vi "Set Toolbar Images.vi"(8 "error in (no error)":errorcluster, 10 "State":T3={"Buttons Displayed"=0, "Button States"=[], "Button Size"=0, "Button Style"=enum."Classic", "Active Button"=0, "Force Regen?"=FALSE, "Tip String Ref"=refnum}) -> (0 "error out":errorcluster, 2 "State Out":T3={"Buttons Displayed"=0, "Button States"=[], "Button Size"=0, "Button Style"=enum."Classic", "Active Button"=0, "Force Regen?"=FALSE, "Tip String Ref"=refnum} caption="State", 3 "Cancelled?":bool)   [LabVIEW 2012, in "Toolbar.xctl"]
doc: "Dialog box to edit the buttons on the toolbar at edit time"
uses:
  Toolbar.xctl
  Toolbar State.ctl
  Button_Class/Button.lvclass
  Button_Class/Type Defs/Button Style.ctl
  Button_Class/Type Defs/Button Status.ctl
  Button_Class/Type Defs/Button Type.ctl
  <vilib>/picture/picture.llb/imagedata.ctl
panel:
  in  "Same Image for all buttons":bool
  out "working Button":refnum<class "Button.lvclass">
  out "Button Images":T1[](array[typedef])
  in  "Button Style":T2 caption="Button Theme"
  in  "Path":path
  in  "Button Sizes":i32
  in  "Current Button":i32
  in  "Buttons Displayed":i32
  in  "Images":enum32{"Off", "Hover", "On", "Disabled"}(tab)
  in  "Paste.Off":bool
  in  "Load.Off":bool
  out "Display.Off":picture
  in  "Paste.Hover":bool
  in  "Load.Hover":bool
  out "Display.Hover":picture
  in  "Paste.On":bool
  in  "Load.On":bool
  out "Display.On":picture
  in  "Paste.Disabled":bool
  in  "Load.Disabled":bool
  out "Display.Disabled":picture
  in  "Type":T4
  in  "Default State":T5
  in  "Cancel":bool
  in  "OK":bool
  # "Toolbar Options"
  # "Button Details"
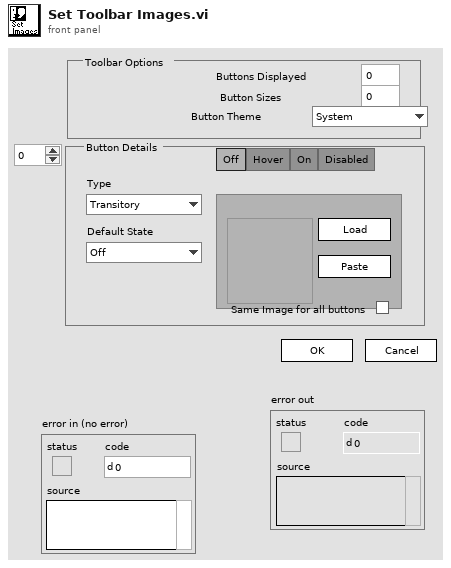
[diagram p1: front panel]
types:
  T1 = typedef "imagedata.ctl" = cluster{"image type":i32, "image depth":i32, "image":u8[], "mask":u8[], "colors":u32[], "Rectangle":cluster{"left":i16, "top":i16, "right":i16, "bottom":i16}}
  T2 = typedef "Button.lvclass/Button Style.ctl" = enum16{"System", "Modern", "Classic", "Rounded", "Silver", "Ni Theme", "Metallic"}
  T3 = typedef "Toolbar.xctl/Toolbar State.ctl" = cluster{"Buttons Displayed":i32, "Button States":refnum<class "Button.lvclass">[], "Button Size":i32, "Button Style":T2, "Active Button":i32, "Force Regen?":bool, "Tip String Ref":refnum<vi>}
  T4 = typedef "Button.lvclass/Button Type.ctl" = enum16{"Transitory", "Latching"}
  T5 = typedef "Button.lvclass/Button Status.ctl" = enum16{"Off", "Hover", "On", "Disabled"}
  T6 = typedef "LVPositionTypeDef.ctl" = cluster{"Left":i32, "Top":i32}
  T7 = typedef "LVBoundsTypeDef.ctl" = cluster{"Width":u32, "Height":u32}
  T8 = enum32{"Page Enabled", "Page Disabled", "Page Disabled & Grayed"}
  T9 = enum32{"existing file", "new file", "new or existing file", "existing dir", "new dir", "new or existing dir", "existing file (use LLBs)", "new file (use LLBs)", "new or existing file (use LLBs)", "new or existing file or directory (use LLBs)", "existing dir (use LLBs)", "new dir (use LLBs)", "new or existing dir (use LLBs)", "existing file or dir", "new file or dir", "new or existing file or dir", "existing file or dir (use LLBs)", "new file or dir (use LLBs)"}
  T10 = typedef "LVRectTypeDef.ctl" = cluster{"left":i16, "top":i16, "right":i16, "bottom":i16}
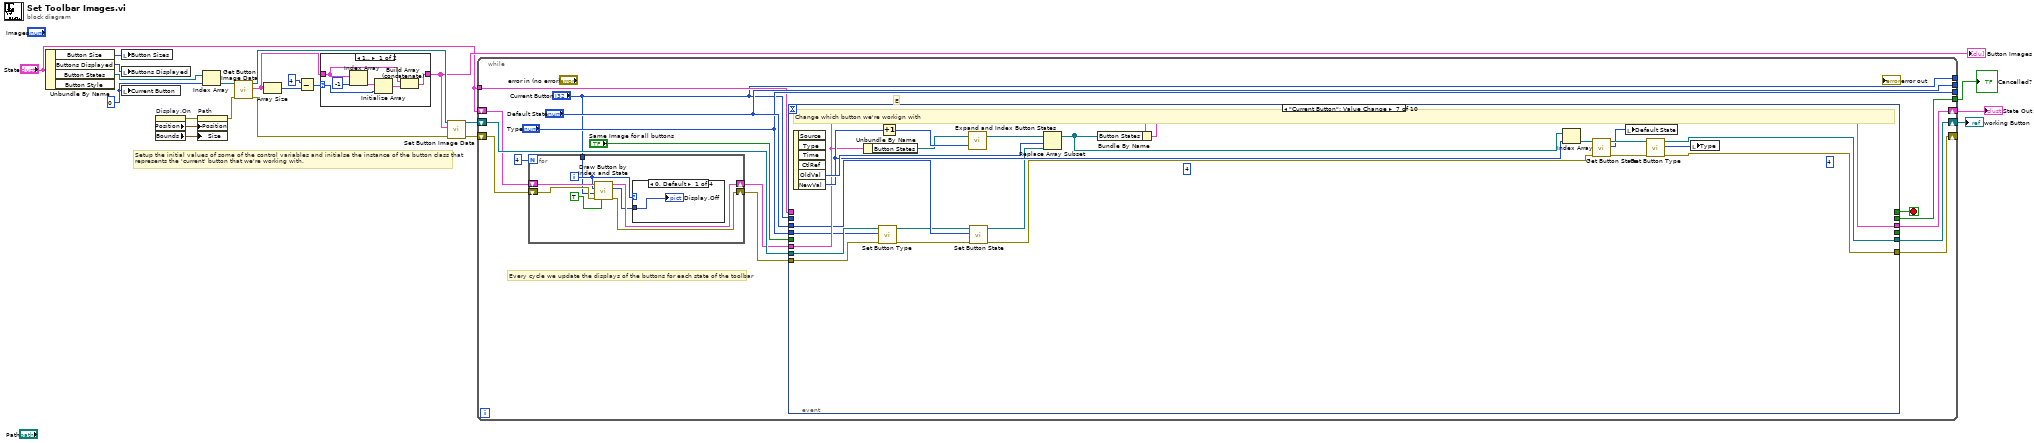
[diagram p0: block diagram]
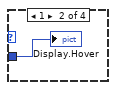
[diagram p3: hidden frame]
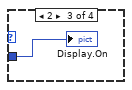
[diagram p4: hidden frame]
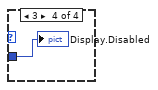
[diagram p5: hidden frame]
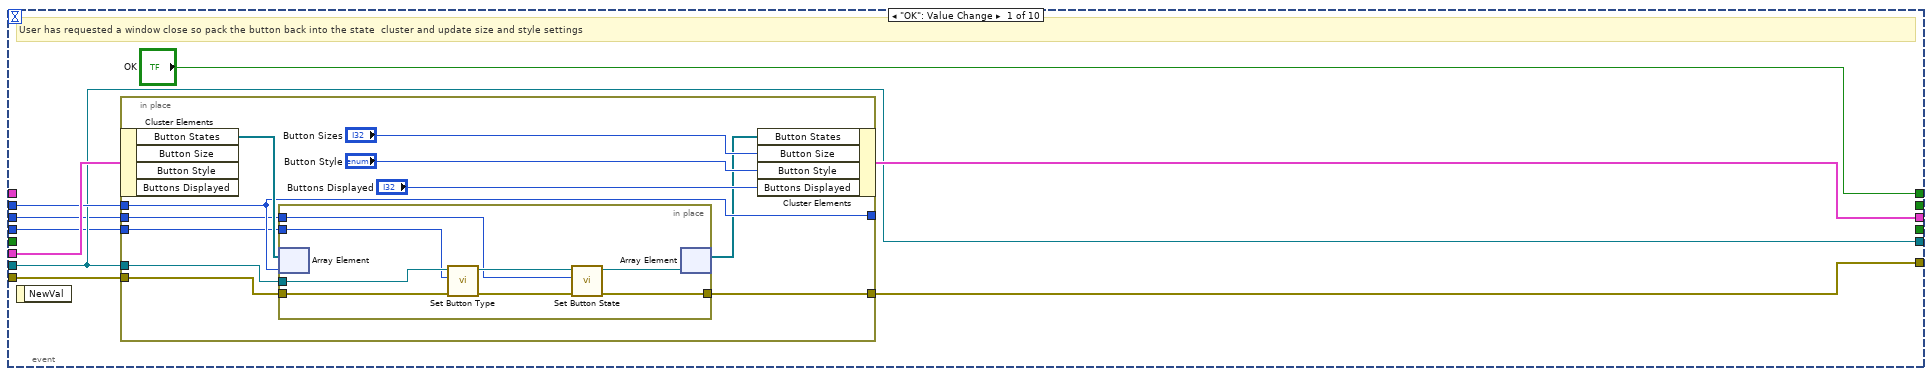
[diagram p6: hidden frame]
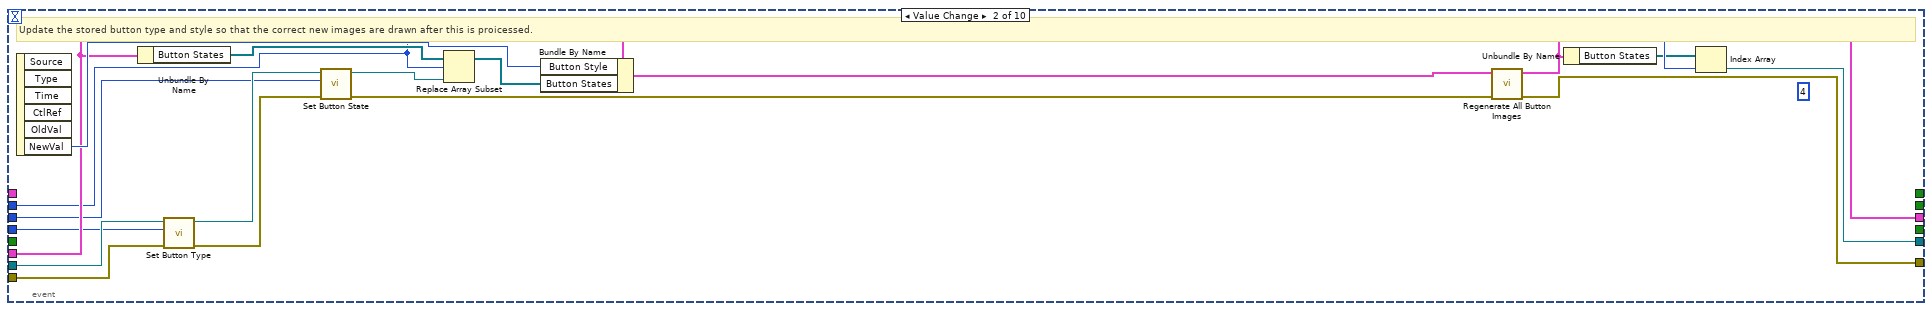
[diagram p7: hidden frame]
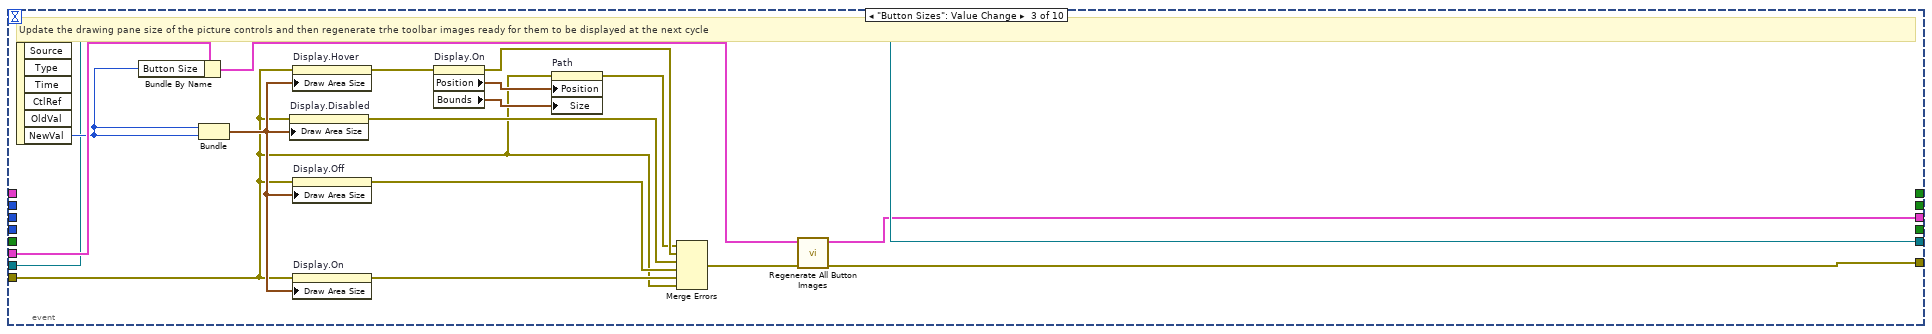
[diagram p8: hidden frame]
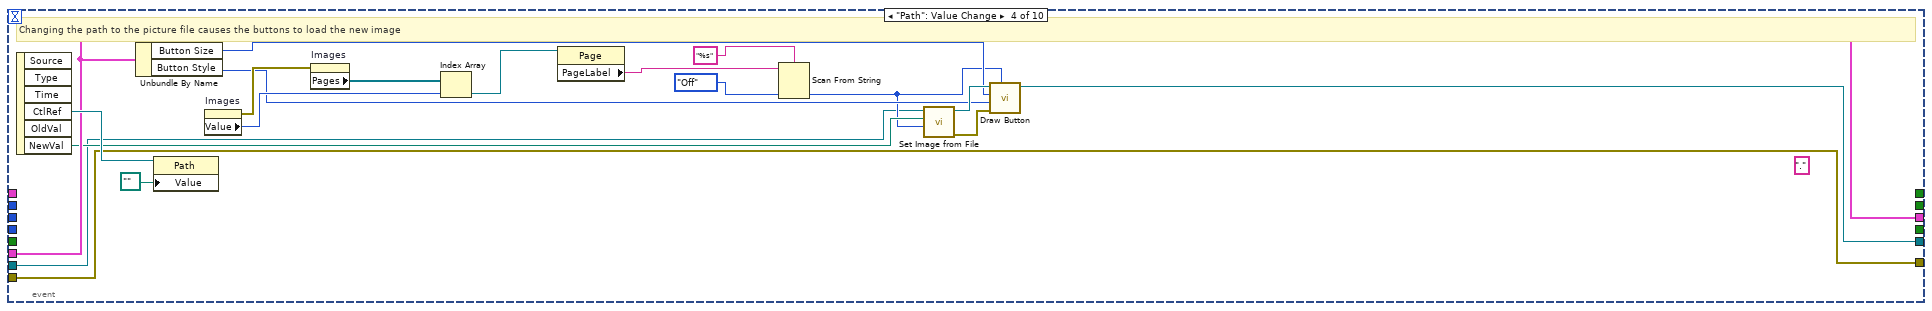
[diagram p9: hidden frame]
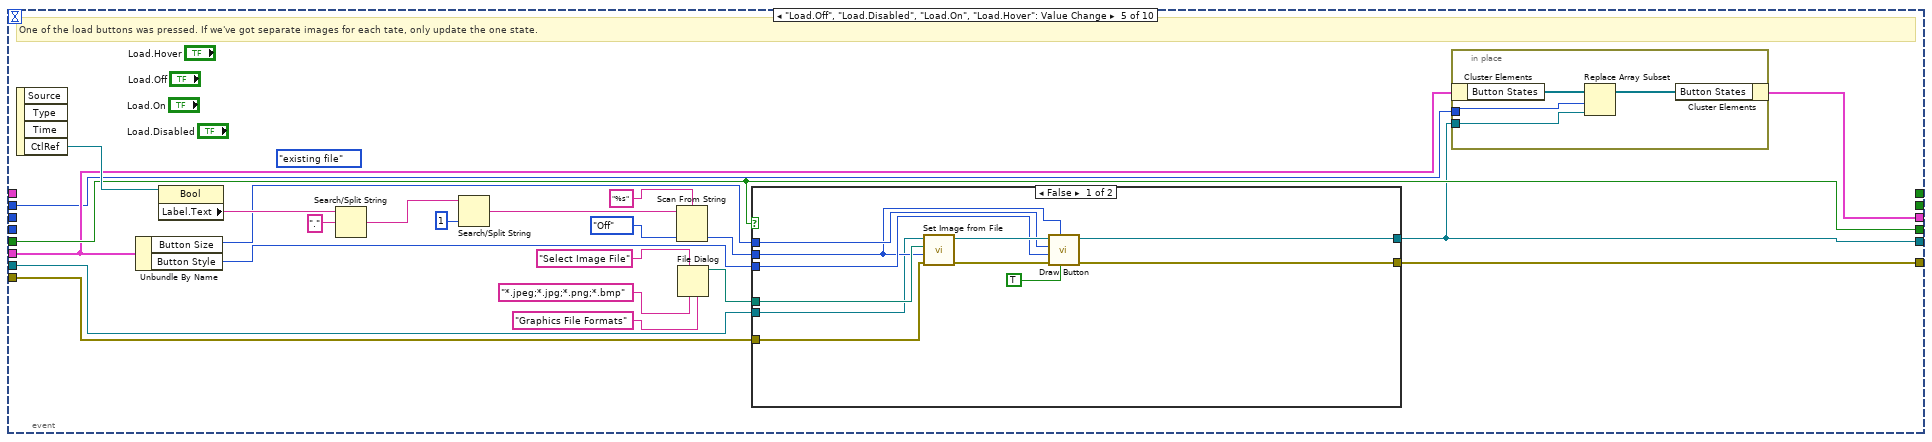
[diagram p10: hidden frame]
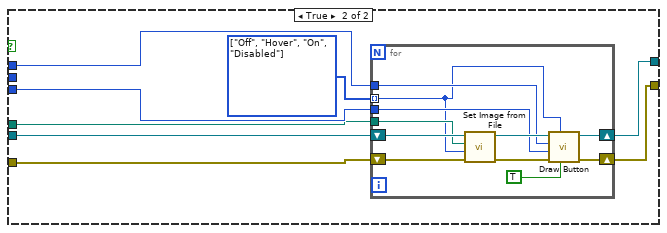
[diagram p11: hidden frame]
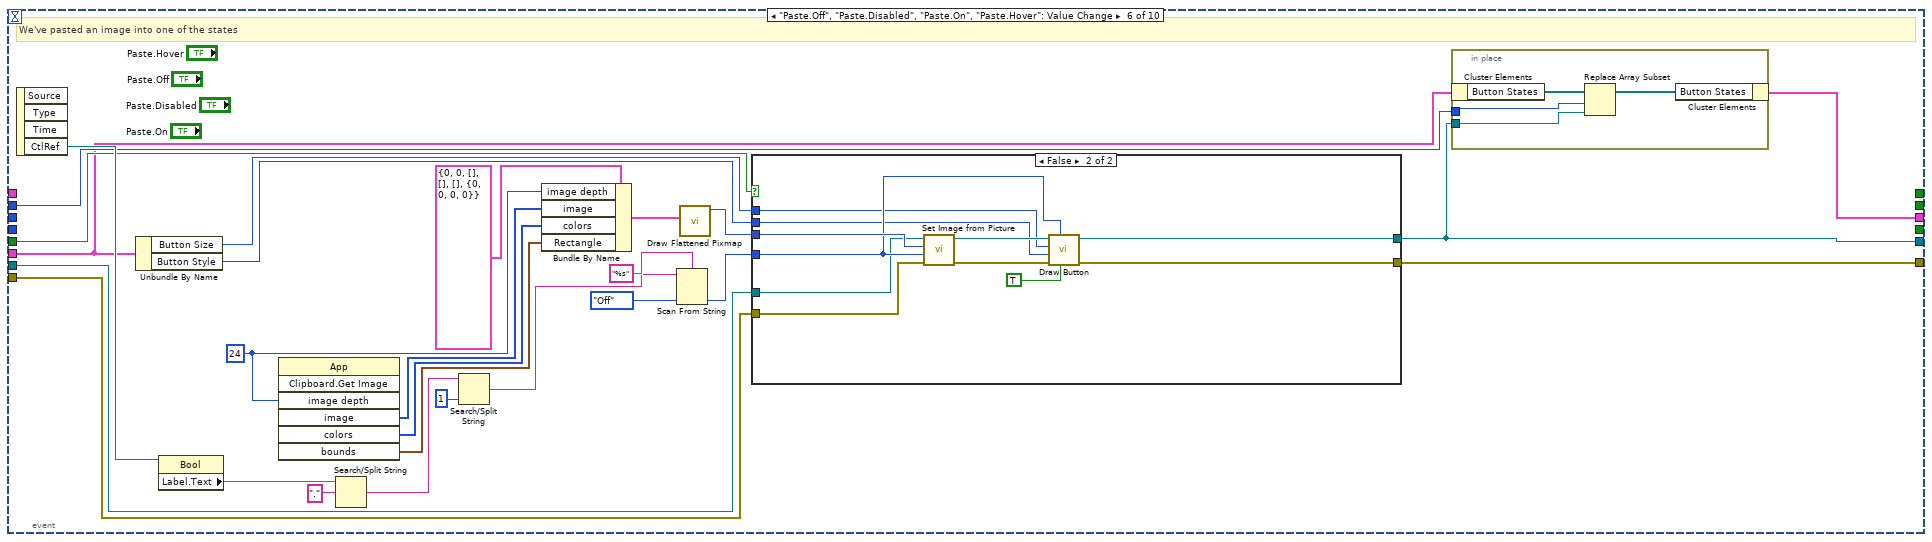
[diagram p12: hidden frame]
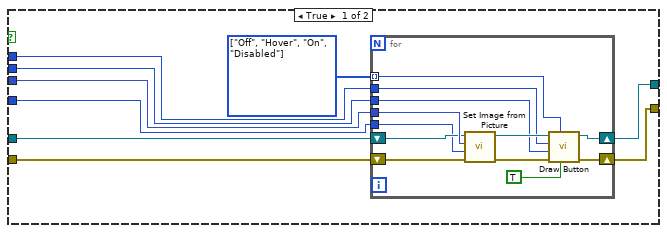
[diagram p13: hidden frame]
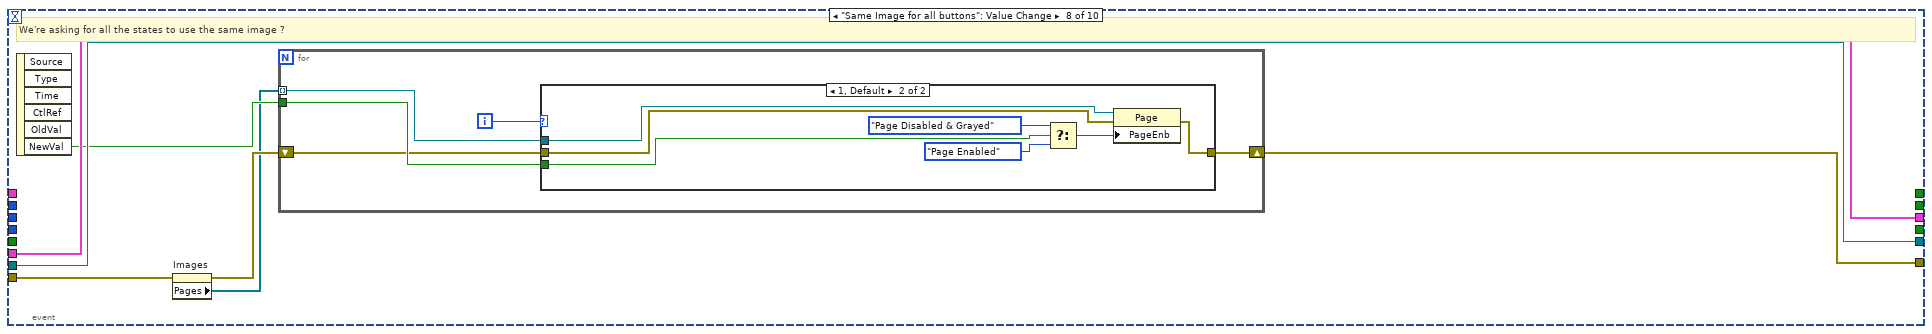
[diagram p14: hidden frame]
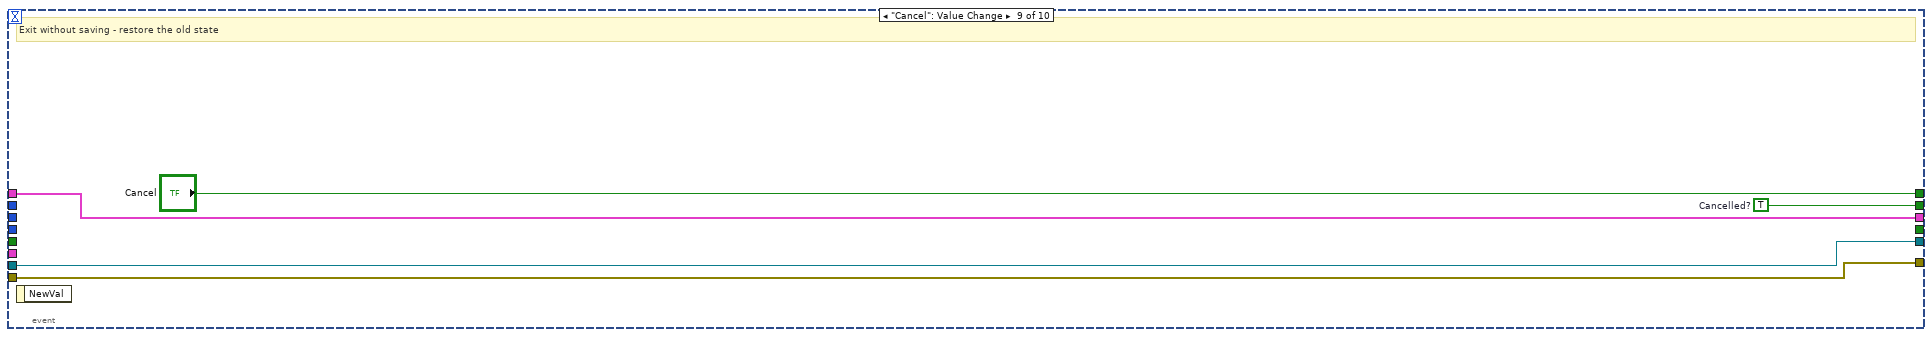
[diagram p16: hidden frame]
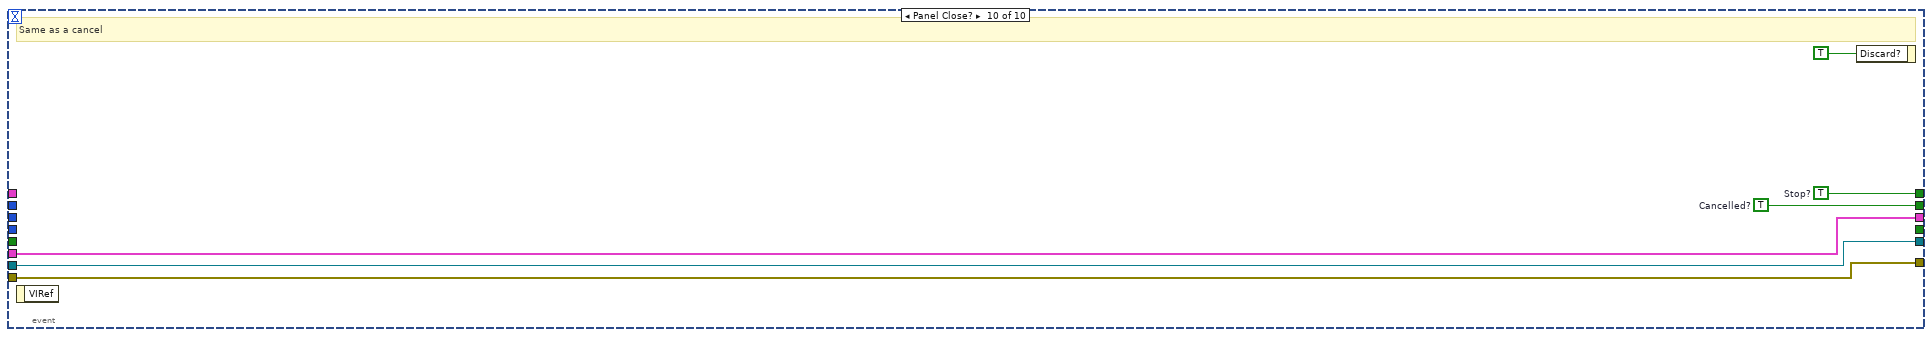
[diagram p17: hidden frame]
diagram:
  w20 = 0 ("Current Button")
  # "Setup the initial values of some of the control variables and initialse the instance of the button class that\nrepresents the 'current' button that we're working with."
  n1 = Unbundle By Name("State") -> ("Button Size"=w19:i32, "Buttons Displayed"=w22:i32, "Button States"=w13:refnum<class "Button.lvclass">[])  [unwired: 1 out]
  n2 = local write "Button Sizes"(w19) -> ()
  n3 = local write "Buttons Displayed"(w22) -> ()
  n4 = local write "Current Button"(w20) -> ()
  n5 = property on="Display.On" class="Pict"() -> (error out=w16:errorcluster, "Position"=w18:T6, "Bounds"=w17:T7)  [unwired: 2 in, 1 out]
  n6 = property on="Path" class="Path"(error in=w16, "Position"=w18, "Size"=w17) -> (error out=w7:errorcluster)  [unwired: 1 in, 1 out]
  n7 = Index Array(array=w13, index=w20) -> (element=w14:refnum<class "Button.lvclass">)
  n8 = call-dynamic "Get Button Image Data.vi"("error in (no error)"=w7, "Button in"=w14) -> ("error out"=w1:errorcluster, "Button Images"=w8:T1[], "Button out"=w15:refnum<class "Button.lvclass">)  [unwired: 7 out]
  n9 = Array Size(array=w8) -> (size(s)=w12:i32)
  n10 = Subtract(x=4 ("Buttons Displayed"), y=w12) -> (x-y=w10:i32)
  n11 = case shown="1.." w10 {
    selector: w10 -> [w27 _]
    tunnel: [w23 w29] -> w9
    tunnel: w8 -> [w25 w29]
    frame 1.. {
      n12 = Index Array(array=w25, index=-1) -> (element=w26:T1)
      n13 = Initialize Array(w26, w27) -> (w24:T1[])
      n14 = Build Array (concatenate)(w25, w24) -> (w23:T1[])
    }
    frame ..0 {
    }
  }
  "Button Images" <- w9
  n15 = call-dynamic "Set Button Image Data.vi"("error in (no error)"=w1, "Button Images"=w9, "Button in"=w15) -> ("error out"=w6:errorcluster, "Button out"=w5:refnum<class "Button.lvclass">)  [unwired: 7 out]
  n16 = while {
    tunnel: [w44] -> w21
    shift-right: [w43] -> w3
    shift-left: "State" -> [w34]
    shift-right: [w42] -> _
    shift-left: w6 -> [w32]
    shift-right: [w40] -> w4
    shift-left: w5 -> [w41]
    tunnel: ["Current Button"] -> _
    tunnel: ["Default State"] -> _
    tunnel: ["Type"] -> _
    tunnel: "State" -> [w35]
    stop <- w45 stop-if-true
    # "Every cycle we update the displays of the buttons for each state of the toolbar"
    # "E"
    n17 = for {
      N: 4 -> [_]
      shift-right: [w52] -> w33
      shift-left: w34 -> [w53]
      shift-right: [w50] -> w31
      shift-left: w32 -> [w51]
      tunnel: "Current Button" -> [w46]
      i -> [w48]
      n18 = call "Draw Button by Index and State.vi"("Force redraw ?"=TRUE, "error in (no error)"=w51, "index"=w46, "Button State"=w48, "State"=w53) -> ("error out"=w50:errorcluster, "Picture Out"=w47:picture, "State out"=w52:T3)  [unwired: 3 in, 1 out]
      n19 = case shown="0, Default" w48 {
        tunnel: w47 -> [w54 w55 w56 w57]
        frame 0, Default {
          "Display.Off" <- w54
        }
        frame 1 {
          "Display.Hover" <- w55
        }
        frame 2 {
          "Display.On" <- w56
        }
        frame 3 {
          "Display.Disabled" <- w57
        }
      }
    }
    n20 = event shown="[6] \"Current Button\": Value Change" {
      selector: _ -> [_ _ _ _ _ _ _ _ _ _]
      dyn-events: _ -> [_ _ _ _ _ _ _ _ _ _]
      timeout: _ -> [_ _ _ _ _ _ _ _ _ _]
      tunnel: ["OK" _ _ _ _ _ _ _ "Cancel" w311] -> w45
      tunnel: [_ _ _ _ _ _ _ _ w306 w310] -> w44
      tunnel: w33 -> [w65 w102 w119 w128 w143 w198 w276 w287 _ w309]
      tunnel: [w64 w89 w104 w128 w142 w197 w277 w287 w302 w309] -> w43
      tunnel: w31 -> [w61 w87 w109 w123 w145 w202 w272 w283 w304 w308]
      tunnel: [w60 w88 w106 w123 w144 w201 w259 w282 w304 w308] -> w42
      tunnel: w41 -> [w62 w97 w114 w122 w147 w204 w271 w288 w303 w307]
      tunnel: [w62 w91 w114 w121 w141 w199 w270 w288 w303 w307] -> w40
      tunnel: "Type" -> [w58 w95 _ _ _ _ w268 _ _ _]
      tunnel: "Default State" -> [w59 w94 _ _ _ _ w269 _ _ _]
      tunnel: "Current Button" -> [w63 w93 _ _ w140 w200 _ _ _ _]
      tunnel: [_ _ _ _ w146 _ _ _ _ _] -> _
      tunnel: "Same Image for all buttons" -> [_ _ _ _ w146 w203 _ _ _ _]
      tunnel: w35 -> [_ _ _ _ _ _ _ _ w302 _]
      event "OK": Value Change {
        # "User has requested a window close so pack the button back into the state  cluster and update size and style settings"
        n21 = event-data() -> ()  [unwired: 2 out]
        n22 = in-place {
          in-place-border: [w76] -> _
          in-place-border: w63 -> [w76]
          in-place-border: w62 -> [w75]
          in-place-border: w61 -> [w74]
          in-place-border: [w73] -> w60
          in-place-border: w59 -> [w68]
          in-place-border: w58 -> [w67]
          n23 = in-place-cluster #1(w65) -> ("Button States"=w77:refnum<class "Button.lvclass">[])  [unwired: 3 out]
          n24 = in-place {
            in-place-border: w75 -> [w83]
            in-place-border: w74 -> [w81]
            in-place-border: [w80] -> w73
            in-place-border: w68 -> [w79]
            in-place-border: w67 -> [w78]
            n25 = in-place-array #2(w77, w76) -> ()  [unwired: 1 out]
            n26 = call-dynamic "Set Button Type.vi"("error in (no error)"=w81, "Type"=w78, "Button in"=w83) -> ("error out"=w85:errorcluster, "Button out"=w84:refnum<class "Button.lvclass">)  [unwired: 7 out]
            n27 = call-dynamic "Set Button State.vi"("error in (no error)"=w85, "State"=w79, "Button in"=w84) -> ("error out"=w80:errorcluster, "Button out"=w82:refnum<class "Button.lvclass">)  [unwired: 7 out]
            n28 = in-place-array #2(w82) -> (w69:refnum<class "Button.lvclass">[])  [unwired: 1 out]
          }
          n29 = in-place-cluster #1("Button States"=w69, "Button Size"="Button Sizes", "Button Style"="Button Style", "Buttons Displayed"="Buttons Displayed") -> (w64:T3)
        }
      }
      event Value Change {
        (unwired) 4
        # "Update the stored button type and style so that the correct new images are drawn after this is proicessed."
        n30 = event-data() -> ("NewVal"=w103:T2)  [unwired: 6 out]
        n31 = Unbundle By Name(w102) -> ("Button States"=w98:refnum<class "Button.lvclass">[])
        n32 = call-dynamic "Set Button Type.vi"("error in (no error)"=w87, "Type"=w95, "Button in"=w97) -> ("error out"=w99:errorcluster, "Button out"=w100:refnum<class "Button.lvclass">)  [unwired: 7 out]
        n33 = call-dynamic "Set Button State.vi"("error in (no error)"=w99, "State"=w94, "Button in"=w100) -> ("error out"=w86:errorcluster, "Button out"=w96:refnum<class "Button.lvclass">)  [unwired: 7 out]
        n34 = Replace Array Subset(array=w98, new element=w96, index=w93) -> (w101:refnum<class "Button.lvclass">[])
        n35 = Bundle By Name(cluster=w102, "Button Style"=w103, "Button States"=w101) -> (w90:T3)
        n36 = call "Regenerate All Button Images.vi"("error in (no error)"=w86, "Display State In in"=w90) -> ("error out"=w88:errorcluster, "Display State In out"=w89:T3)  [unwired: 8 in]
        n37 = Unbundle By Name(w89) -> ("Button States"=w92:refnum<class "Button.lvclass">[])
        n38 = Index Array(array=w92, index=w93) -> (element=w91:refnum<class "Button.lvclass">)
      }
      event "Button Sizes": Value Change {
        # "Update the drawing pane size of the picture controls and then regenerate trhe toolbar images ready for them to be displayed at the next cycle"
        n39 = event-data() -> ("NewVal"=w115:i32)  [unwired: 6 out]
        n40 = Bundle By Name(cluster=w119, "Button Size"=w115) -> (w105:T3)
        n41 = Bundle("NewVal"=w115, "NewVal"=w115) -> (w120:cluster{"NewVal":i32, "NewVal":i32})  [unwired: 1 out]
        n42 = property on="Display.Disabled" class="Pict"(error in=w109, "Draw Area Size"=w120) -> (error out=w111:errorcluster)  [unwired: 1 in, 1 out]
        n43 = property on="Display.Hover" class="Pict"(error in=w109, "Draw Area Size"=w120) -> (error out=w116:errorcluster)  [unwired: 1 in, 1 out]
        n44 = property on="Display.Off" class="Pict"(error in=w109, "Draw Area Size"=w120) -> (error out=w112:errorcluster)  [unwired: 1 in, 1 out]
        n45 = property on="Display.On" class="Pict"(error in=w109, "Draw Area Size"=w120) -> (error out=w113:errorcluster)  [unwired: 1 in, 1 out]
        n46 = property on="Display.On" class="Pict"(error in=w116) -> (error out=w110:errorcluster, "Position"=w117:T6, "Bounds"=w118:T7)  [unwired: 1 in, 1 out]
        n47 = property on="Path" class="Path"(error in=w109, "Position"=w117, "Size"=w118) -> (error out=w108:errorcluster)  [unwired: 1 in, 1 out]
        n48 = Merge Errors(w108, w110, w111, w112, w113, w109) -> (w107:errorcluster)
        n49 = call "Regenerate All Button Images.vi"("error in (no error)"=w107, "Display State In in"=w105) -> ("error out"=w106:errorcluster, "Display State In out"=w104:T3)  [unwired: 8 in]
      }
      event "Path": Value Change {
        (unwired) "." ("search string/char (-)")
        # "Changing the path to the picture file causes the buttons to load the new image"
        n50 = event-data() -> ("CtlRef"=w134:refnum<vi>, "NewVal"=w127:path)  [unwired: 5 out]
        n51 = Unbundle By Name(w128) -> ("Button Size"=w126:i32, "Button Style"=w125:T2)
        n52 = property class="Path"(reference=w134, "Value"=path "") -> ()  [unwired: 1 in, 2 out]
        n53 = property on="Images" class="TabCtl (strict)"() -> (error out=w136:errorcluster, "Value"=w137:enum32{"Off", "Hover", "On", "Disabled"})  [unwired: 2 in, 1 out]
        n54 = property on="Images" class="TabCtl (strict)"(error in=w136) -> ("Pages"=w138:refnum<vi>[])  [unwired: 1 in, 2 out]
        n55 = Index Array(array=w138, index=w137) -> (element=w135:refnum<vi>)
        n56 = property class="Page"(reference=w135) -> ("PageLabel"=w131:string)  [unwired: 1 in, 2 out]
        n57 = Scan From String(format string="%s", input string=w131, default 1=Button_Status."Off" ("Button State")) -> (output 1=w124:T5)  [unwired: 2 in, 3 out]
        n58 = call-dynamic "Set Image from File.vi"("State"=w124, "path"=w127, "Button in"=w122) -> ("error out"=w129:errorcluster, "Button out"=w130:refnum<class "Button.lvclass">)  [unwired: 1 in, 6 out]
        n59 = call "Draw Button.vi"("Button State"=w124, "error in (no error)"=w129, "Button Style"=w125, "Button Size"=w126, "Button.lvclass"=w130) -> ("Button.lvclass Out"=w121:refnum<class "Button.lvclass">)  [unwired: 1 in, 5 out]
      }
      event "Load.Off", "Load.Disabled", "Load.On", "Load.Hover": Value Change {
        (unwired) T9."existing file" ("select mode (2)")
        # "One of the load buttons was pressed. If we've got separate images for each tate, only update the one state."
        n60 = event-data() -> ("CtlRef"=w162:refnum<vi>)  [unwired: 4 out]
        n61 = Unbundle By Name(w143) -> ("Button Size"=w150:i32, "Button Style"=w149:T2)
        n62 = property class="Bool"(reference=w162) -> ("Label.Text"=w152:string)  [unwired: 1 in, 2 out]
        n63 = Search/Split String(string=w152, search string/char (-)=".") -> (match + rest of string=w157:string)  [unwired: 3 out]
        n64 = Search/Split String(string=w157, offset (0)=1) -> (match + rest of string=w153:string)  [unwired: 3 out]
        n65 = Scan From String(format string="%s", input string=w153, default 1=Button_Status."Off" ("Button State")) -> (output 1=w148:T5)  [unwired: 2 in, 3 out]
        n66 = File Dialog(4:"Graphics File Formats" ("pattern label"), 6:"*.jpeg;*.jpg;*.png;*.bmp" ("pattern"), 7:"Select Image File" ("prompt")) -> (3:w151:path)  [unwired: 1 in, 6 out]
        n67 = case shown="False" w146 {
          tunnel: w151 -> [w177 w178]
          tunnel: w150 -> [w174 w180]
          tunnel: w149 -> [w173 w181]
          tunnel: w148 -> [w172 _]
          tunnel: w147 -> [w171 w182]
          tunnel: [w170 w183] -> w141
          tunnel: w145 -> [w169 w185]
          tunnel: [w168 w184] -> w144
          frame False {
            n68 = call-dynamic "Set Image from File.vi"("error in (no error)"=w169, "State"=w172, "path"=w177, "Button in"=w171) -> ("error out"=w175:errorcluster, "Button out"=w176:refnum<class "Button.lvclass">)  [unwired: 6 out]
            n69 = call "Draw Button.vi"("Force redraw ?"=TRUE, "Button State"=w172, "error in (no error)"=w175, "Button Style"=w173, "Button Size"=w174, "Button.lvclass"=w176) -> ("error out"=w168:errorcluster, "Button.lvclass Out"=w170:refnum<class "Button.lvclass">)  [unwired: 4 out]
          }
          frame True {
            w179 = T5[] [enum."Off", enum."Hover", enum."On", enum."Disabled"] items=["Off", "Hover", "On", "Disabled"]
            n70 = for {
              shift-right: [w193] -> w184
              shift-left: w185 -> [w194]
              shift-right: [w192] -> w183
              shift-left: w182 -> [w191]
              tunnel: w181 -> [w190]
              tunnel: w180 -> [w189]
              tunnel: w179 -> [w187] mode=indexing
              tunnel: w178 -> [w188]
              n71 = call-dynamic "Set Image from File.vi"("error in (no error)"=w194, "State"=w187, "path"=w188, "Button in"=w191) -> ("error out"=w195:errorcluster, "Button out"=w196:refnum<class "Button.lvclass">)  [unwired: 6 out]
              n72 = call "Draw Button.vi"("Force redraw ?"=TRUE, "Button State"=w187, "error in (no error)"=w195, "Button Style"=w190, "Button Size"=w189, "Button.lvclass"=w196) -> ("error out"=w193:errorcluster, "Button.lvclass Out"=w192:refnum<class "Button.lvclass">)  [unwired: 4 out]
            }
          }
        }
        n73 = in-place {
          in-place-border: w140 -> [w164]
          in-place-border: w141 -> [w163]
          n74 = in-place-cluster #3(w143) -> ("Button States"=w166:refnum<class "Button.lvclass">[])
          n75 = Replace Array Subset(array=w166, new element=w163, index=w164) -> (w165:refnum<class "Button.lvclass">[])
          n76 = in-place-cluster #3("Button States"=w165) -> (w142:T3)
        }
      }
      event "Paste.Off", "Paste.Disabled", "Paste.On", "Paste.Hover": Value Change {
        w218 = 24 ("Image Depth")
        # "We've pasted an image into one of the states"
        n77 = event-data() -> ("CtlRef"=w222:refnum<vi>)  [unwired: 4 out]
        n78 = Unbundle By Name(w198) -> ("Button Size"=w206:i32, "Button Style"=w205:T2)
        n79 = property class="Bool"(reference=w222) -> ("Label.Text"=w221:string)  [unwired: 1 in, 2 out]
        n80 = invoke class="App" method="Clipboard.Get Image"("image depth"=w218) -> ("image"=w217:u8[], "colors"=w216:u32[], "bounds"=w215:T10)  [unwired: 6 in, 4 out]
        n81 = Search/Split String(string=w221, search string/char (-)=".") -> (match + rest of string=w214:string)  [unwired: 3 out]
        n82 = Search/Split String(string=w214, offset (0)=1) -> (match + rest of string=w210:string)  [unwired: 3 out]
        n83 = Bundle By Name(cluster=T1 {"image type"=0, "image depth"=0, "image"=[], "mask"=[], "colors"=[], "Rectangle"={"left"=0, "top"=0, "right"=0, "bottom"=0}} ("image data"), "image depth"=w218, "image"=w217, "colors"=w216, "Rectangle"=w215) -> (w209:T1)
        n84 = Scan From String(format string="%s", input string=w210, default 1=Button_Status."Off" ("Button State")) -> (output 1=w207:T5)  [unwired: 2 in, 3 out]
        n85 = call <vilib>:"Draw Flattened Pixmap.vi"("image data"=w209) -> ("new picture"=w208:picture)  [unwired: 1 in, 7 out]
        n86 = case shown="False" w203 {
          tunnel: w208 -> [w235 w258]
          tunnel: w207 -> [w234 w255]
          tunnel: w206 -> [w233 w254]
          tunnel: w205 -> [w232 w253]
          tunnel: w204 -> [w231 w252]
          tunnel: [w230 w251] -> w199
          tunnel: w202 -> [w228 w250]
          tunnel: [w227 w249] -> w201
          frame True {
            w229 = T5[] [enum."Off", enum."Hover", enum."On", enum."Disabled"] items=["Off", "Hover", "On", "Disabled"]
            n87 = for {
              tunnel: w235 -> [w247]
              tunnel: w234 -> [w240]
              tunnel: w233 -> [w244]
              tunnel: w232 -> [w243]
              tunnel: w229 -> [w239] mode=indexing
              shift-right: [w241] -> w230
              shift-left: w231 -> [w242]
              shift-right: [w237] -> w227
              shift-left: w228 -> [w238]
              n88 = call-dynamic "Set Image from Picture.vi"("error in (no error)"=w238, "State"=w240, "Picture"=w247, "Button in"=w242) -> ("error out"=w246:errorcluster, "Button out"=w245:refnum<class "Button.lvclass">)  [unwired: 1 in, 5 out]
              n89 = call "Draw Button.vi"("Force redraw ?"=TRUE, "Button State"=w239, "error in (no error)"=w246, "Button Style"=w243, "Button Size"=w244, "Button.lvclass"=w245) -> ("error out"=w237:errorcluster, "Button.lvclass Out"=w241:refnum<class "Button.lvclass">)  [unwired: 4 out]
            }
          }
          frame False {
            n90 = call-dynamic "Set Image from Picture.vi"("error in (no error)"=w250, "State"=w255, "Picture"=w258, "Button in"=w252) -> ("error out"=w257:errorcluster, "Button out"=w256:refnum<class "Button.lvclass">)  [unwired: 1 in, 5 out]
            n91 = call "Draw Button.vi"("Force redraw ?"=TRUE, "Button State"=w255, "error in (no error)"=w257, "Button Style"=w253, "Button Size"=w254, "Button.lvclass"=w256) -> ("error out"=w249:errorcluster, "Button.lvclass Out"=w251:refnum<class "Button.lvclass">)  [unwired: 4 out]
          }
        }
        n92 = in-place {
          in-place-border: w200 -> [w224]
          in-place-border: w199 -> [w223]
          n93 = in-place-cluster #4(w198) -> ("Button States"=w226:refnum<class "Button.lvclass">[])
          n94 = Replace Array Subset(array=w226, new element=w223, index=w224) -> (w225:refnum<class "Button.lvclass">[])
          n95 = in-place-cluster #4("Button States"=w225) -> (w197:T3)
        }
      }
      event "Current Button": Value Change {
        (unwired) 4 ("Buttons Displayed")
        (unwired) 4
        # "Change which button we're workign with"
        n96 = event-data() -> ("OldVal"=w280:i32, "NewVal"=w279:i32)  [unwired: 5 out]
        n97 = Unbundle By Name(w276) -> ("Button States"=w274:refnum<class "Button.lvclass">[])
        n98 = call-dynamic "Set Button Type.vi"("error in (no error)"=w272, "Type"=w268, "Button in"=w271) -> ("error out"=w266:errorcluster, "Button out"=w267:refnum<class "Button.lvclass">)  [unwired: 7 out]
        n99 = Increment(x=w279) -> (x+1=w278:i32)
        n100 = call "Expand and Index Button States.vi"("Button Index"=w278, "Button States"=w274) -> ("Button States Out"=w275:refnum<class "Button.lvclass">[])  [unwired: 1 out]
        n101 = call-dynamic "Set Button State.vi"("error in (no error)"=w266, "State"=w269, "Button in"=w267) -> ("error out"=w273:errorcluster, "Button out"=w265:refnum<class "Button.lvclass">)  [unwired: 7 out]
        n102 = Replace Array Subset(array=w275, new element=w265, index=w280) -> (w281:refnum<class "Button.lvclass">[])
        n103 = Bundle By Name(cluster=w276, "Button States"=w281) -> (w277:T3)
        n104 = Index Array(array=w281, index=w279) -> (element=w264:refnum<class "Button.lvclass">)
        n105 = call-dynamic "Get Button State.vi"("error in (no error)"=w273, "Button in"=w264) -> ("error out"=w260:errorcluster, "State"=w262:T5, "Button out"=w263:refnum<class "Button.lvclass">)  [unwired: 7 out]
        n106 = local write "Default State"(w262) -> ()
        n107 = call-dynamic "Get Button Type.vi"("error in (no error)"=w260, "Button in"=w263) -> ("error out"=w259:errorcluster, "Type"=w261:T4, "Button out"=w270:refnum<class "Button.lvclass">)  [unwired: 7 out]
        n108 = local write "Type"(w261) -> ()
      }
      event "Same Image for all buttons": Value Change {
        # "We're asking for all the states to use the same image ?"
        n109 = event-data() -> ("NewVal"=w285:bool)  [unwired: 6 out]
        n110 = property on="Images" class="TabCtl (strict)"(error in=w283) -> (error out=w286:errorcluster, "Pages"=w284:refnum<vi>[])  [unwired: 1 in, 1 out]
        n111 = for {
          shift-right: [w289] -> w282
          shift-left: w286 -> [w290]
          tunnel: w285 -> [w292]
          tunnel: w284 -> [w291] mode=indexing
          i -> [w293]
          n112 = case shown="1, Default" w293 {
            tunnel: w292 -> [_ w296]
            tunnel: w291 -> [_ w301]
            tunnel: w290 -> [w294 w300]
            tunnel: [w294 w299] -> w289
            frame 0 {
            }
            frame 1, Default {
              n113 = Select(t=T8."Page Disabled & Grayed" ("Page Enabled State"), s=w296, f=T8."Page Enabled" ("Page Enabled State")) -> (s? t:f=w295:T8)
              n114 = property class="Page"(reference=w301, error in=w300, "PageEnb"=w295) -> (error out=w299:errorcluster)  [unwired: 1 out]
            }
          }
        }
      }
      event "Cancel": Value Change {
        w306 = TRUE  # Cancelled?
        # "Exit without saving - restore the old state"
        n115 = event-data() -> ()  [unwired: 2 out]
      }
      event Panel Close? {
        w310 = TRUE  # Cancelled?
        w311 = TRUE  # Stop?
        # "Same as a cancel"
        n116 = event-data() -> ()  [unwired: 2 out]
        n117 = event-data("Discard?"=TRUE) -> ()  [unwired: 1 in, 1 out]
      }
    }
  }
  "Cancelled?" <- w21
  "State Out" <- w3
  "working Button" <- w4
